vi "Set Tool Title.vi"(8 "error in":errorcluster, 10 "title":string, 11 "tool entry":string) -> (0 "error out":errorcluster, 3 "tool entry out":string)   [LabVIEW 2020, in "MCP Server.lvlib"]
doc: "Sets the title of a tools/list entry, for Complete Tool Entry.vi. The entry's title is replaced by title. When title is empty the entry has no title. With an error in the entry is passed through."
uses:
  MCP Server.lvlib
  c7e9b049-486c-4beb-b028-b11b7492152b.vi
  <vilib>/JDP Science/JSONtext/Variant to JSON Text.vi
  <vilib>/JDP Science/JSONtext/support/Format JSON Object.vi
  <vilib>/JDP Science/JSONtext/LVClass Serializer/JSONtext LVClass Serializer.lvclass
  <vilib>/JDP Science/JSONtext/JSONtext.lvlib
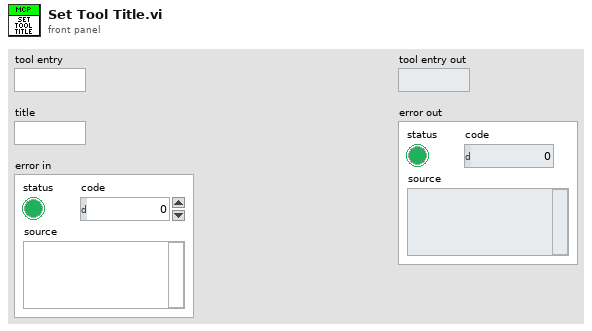
[diagram p1: front panel]
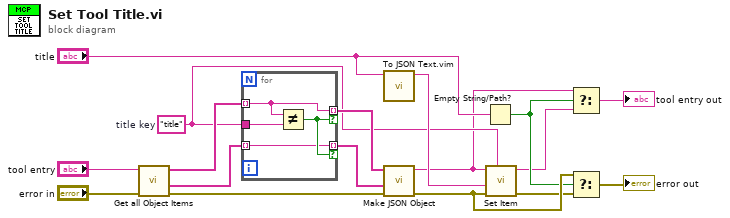
[diagram p0: block diagram]
diagram:
  w8 = "title"  # title key
  n1 = call <vilib>:"Get all Object Items.vi"("error in (no error)"="error in", "JSON"="tool entry") -> ("error out"=w10:errorcluster, "<JSON>"=w13:string[], "Item Names"=w14:string[])  [unwired: 6 in, 1 out]
  n2 = for {
    tunnel: w14 -> [w20] mode=indexing
    tunnel: w13 -> [w18] mode=indexing
    tunnel: w8 -> [w21]
    tunnel: [w20] -> w12 mode=indexing if=w19
    tunnel: [w18] -> w11 mode=indexing if=w19
    n3 = Not Equal?(x=w20, y=w21) -> (x != y?=w19:bool)
  }
  n4 = call "To JSON Text.vim"("Anything"="title") -> ("<JSON>"=w9:string)  [unwired: 9 in, 1 out]
  n5 = call <vilib>:"Make JSON Object.vi"("error in (no error)"=w10, "JSON Items"=w11, "Item Names"=w12) -> ("error out"=w7:errorcluster, "<JSON>"=w5:string)  [unwired: 7 in]
  n6 = Empty String/Path?(string/path="title") -> (empty?=w4:bool)
  n7 = call <vilib>:"Set Item.vi"("$Path or Item Name"=w8, "error in (no error)"=w7, "JSON to Insert"=w9, "JSON"=w5) -> ("error out"=w6:errorcluster, "<JSON>"=w3:string)  [unwired: 4 in, 1 out]
  n8 = Select(t=w5, s=w4, f=w3) -> (s? t:f=→"tool entry out":string)
  n9 = Select(t=w7, s=w4, f=w6) -> (s? t:f=→"error out":errorcluster)
